vi "Get_Diagnostics.vi"(8 "error in (no error)":errorcluster, 11 "Motor in":refnum<class "Motor.lvclass">) -> (0 "error out":errorcluster, 2 "Diagnostics":T1, 3 "Motor out":refnum<class "Motor.lvclass">)   [LabVIEW 2021, in "Motor.lvclass"]
uses:
  Motor.lvclass
  Motor.lvclass/Motor.ctl
  ServoDrive/ServoDrive.lvclass
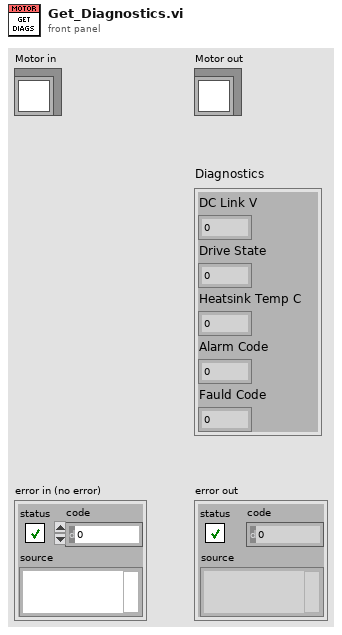
[diagram p1: front panel]
types:
  T1 = cluster{"DC Link V":dbl, "Drive State":u16, "Heatsink Temp C":dbl, "Alarm Code":dbl, "Fauld Code":dbl}
  T2 = cluster{"Fauld Code":dbl, "Alarm Code":dbl, "Drive State":u16, "DC Link V":dbl, "Heatsink Temp C":dbl}
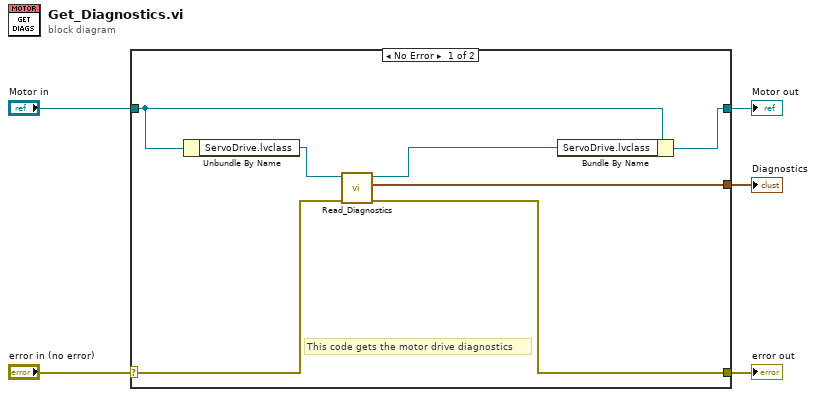
[diagram p0: block diagram]
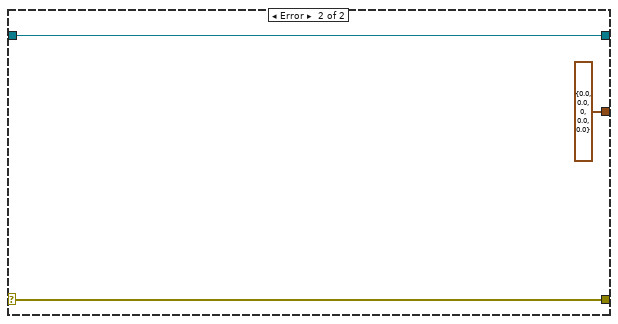
[diagram p2: hidden frame]
diagram:
  n1 = case shown="No Error" "error in (no error)" {
    selector: "error in (no error)" -> [w9 w15]
    tunnel: [w8 w15] -> w4
    tunnel: [w11 w14] -> w2
    tunnel: "Motor in" -> [w12 w14]
    tunnel: [w6 T2 {"Fauld Code"=0.0, "Alarm Code"=0.0, "Drive State"=0, "DC Link V"=0.0, "Heatsink Temp C"=0.0} ("Diagnostics")] -> w1
    frame No Error {
      # "This code gets the motor drive diagnostics"
      n2 = Unbundle By Name(w12) -> ("ServoDrive.lvclass"=w10:refnum<class "ServoDrive.lvclass">)
      n3 = call-dynamic "Read_Diagnostics.vi"("error in (no error)"=w9, "ServoDrive in"=w10) -> ("error out"=w8:errorcluster, "Diagnostics"=w6:T1, "ServoDrive out"=w7:refnum<class "ServoDrive.lvclass">)  [unwired: 7 in]
      n4 = Bundle By Name(cluster=w12, "ServoDrive.lvclass"=w7) -> (w11:refnum<class "Motor.lvclass">)
    }
    frame Error {
    }
  }
  "error out" <- w4
  "Motor out" <- w2
  "Diagnostics" <- w1
